vi "NanonisGetZValue.vi"(8 "error in (no error)":errorcluster, 11 "String input":string="string test") -> (0 "error out":errorcluster, 3 "String output":string)   [LabVIEW 2011]
uses:
  <userlib>/Nanonis Prog Interface/Nanonis Prog Interface.lvlib
panel:
  out "Z position (m)":sgl format="%#_6p"
  out "Application ref out":refnum<vi>
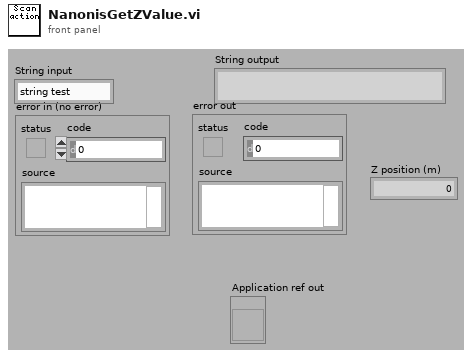
[diagram p1: front panel]
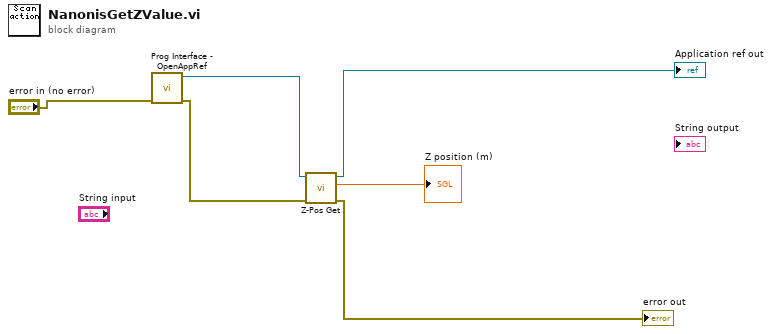
[diagram p0: block diagram]
diagram:
  n1 = call <userlib>:"Prog Interface - OpenAppRef.vi"("Error in (no error)"="error in (no error)") -> ("Error out"=w4:errorcluster, "Application reference"=w5:refnum<vi>)  [unwired: 5 in]
  n2 = call <userlib>:"Z-Pos Get.vi"("error in (no error)"=w4, "Application ref in"=w5) -> ("error out"=→"error out":errorcluster, "Z position (m)"=→"Z position (m)":sgl, "Application ref out"=→"Application ref out":refnum<vi>)  [unwired: 7 in]
